vi "Update.vi"(8 "error in (no error)":errorcluster, 11 "Deck in":refnum<class "Deck.lvclass">) -> (0 "error out":errorcluster, 2 "Audio Block":dbl[][](array[numeric]), 3 "Deck out":refnum<class "Deck.lvclass">)   [LabVIEW 2019, in "Deck.lvclass"]
uses:
  Deck.lvclass
  Deck.lvclass/Deck.ctl
  State.ctl
  Packed Libraries/Globals.lvlibp/Constants.vi
  <vilib>/gmath/NI_Gmath.lvlib
  Libraries/User Interface/User Interface.lvlib
  Packed Libraries/Messaging.lvlibp
  Packed Libraries/Globals.lvlibp
  Packed Libraries/Audio Processing.lvlibp
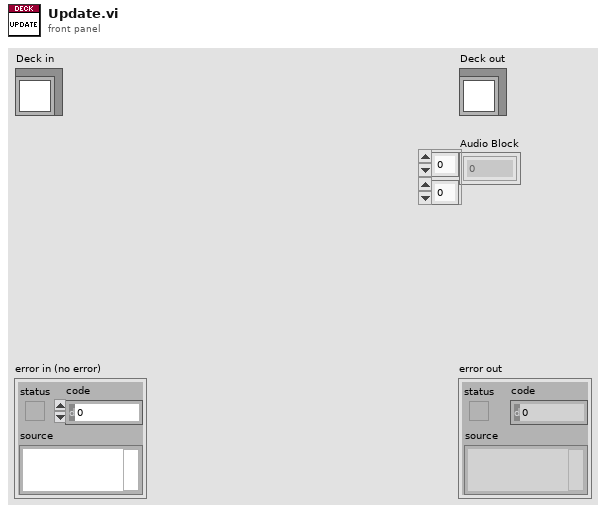
[diagram p1: front panel]
types:
  T1 = typedef "Deck.lvclass/State.ctl" = enum16{"No Track", "Loading", "Active", "Scratching", "Brake", "Backspin"}
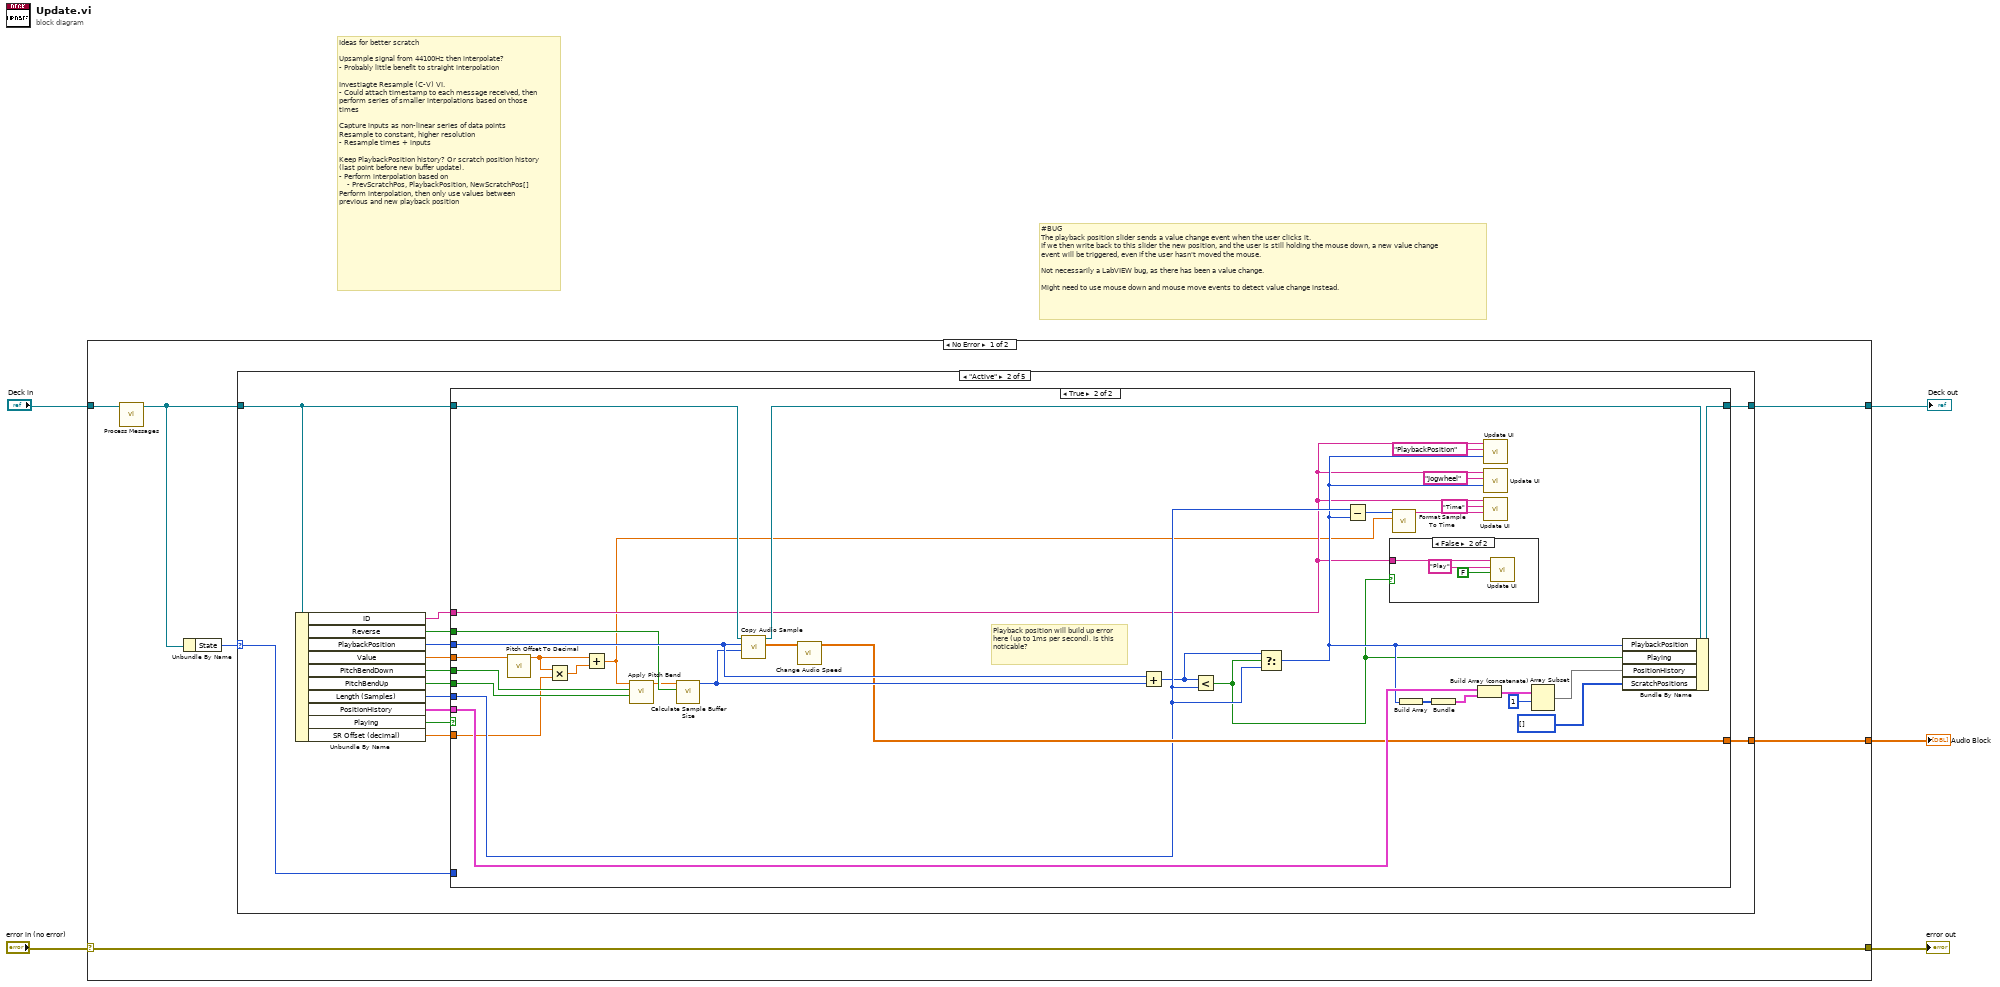
[diagram p0: block diagram]
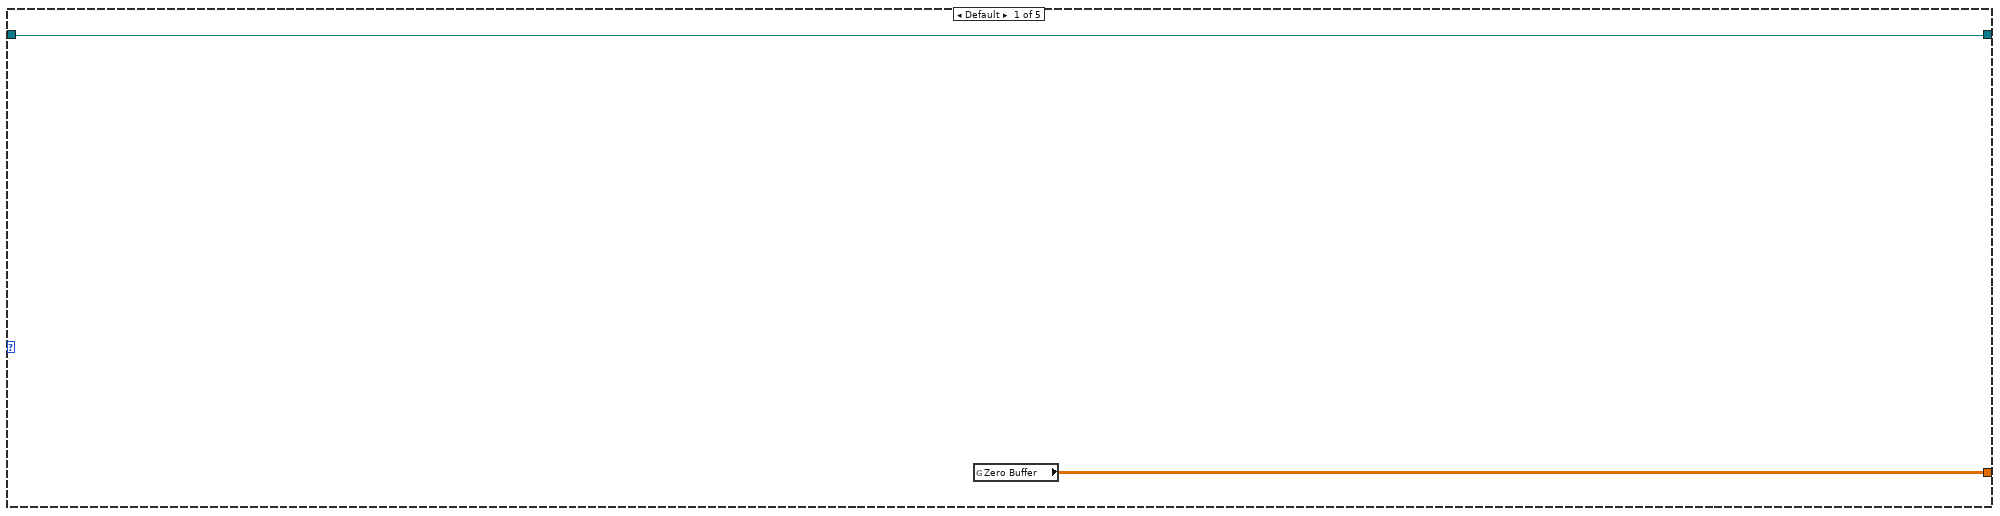
[diagram p2: hidden frame]
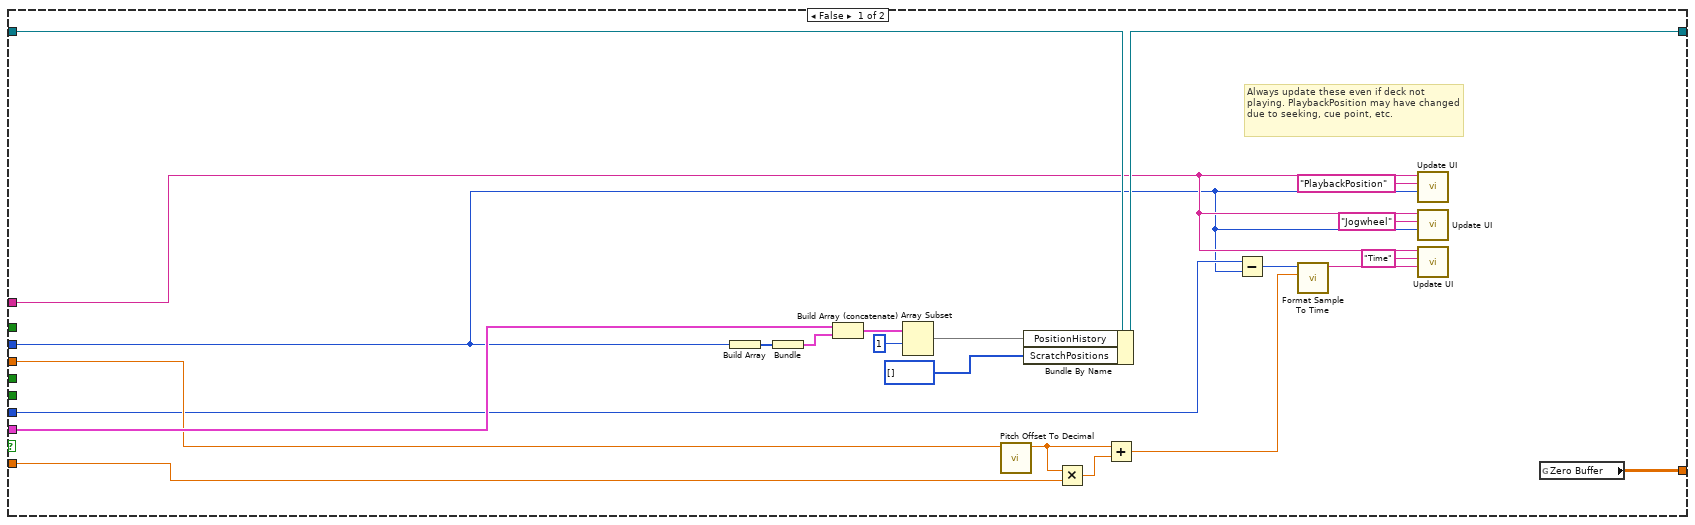
[diagram p3: hidden frame]
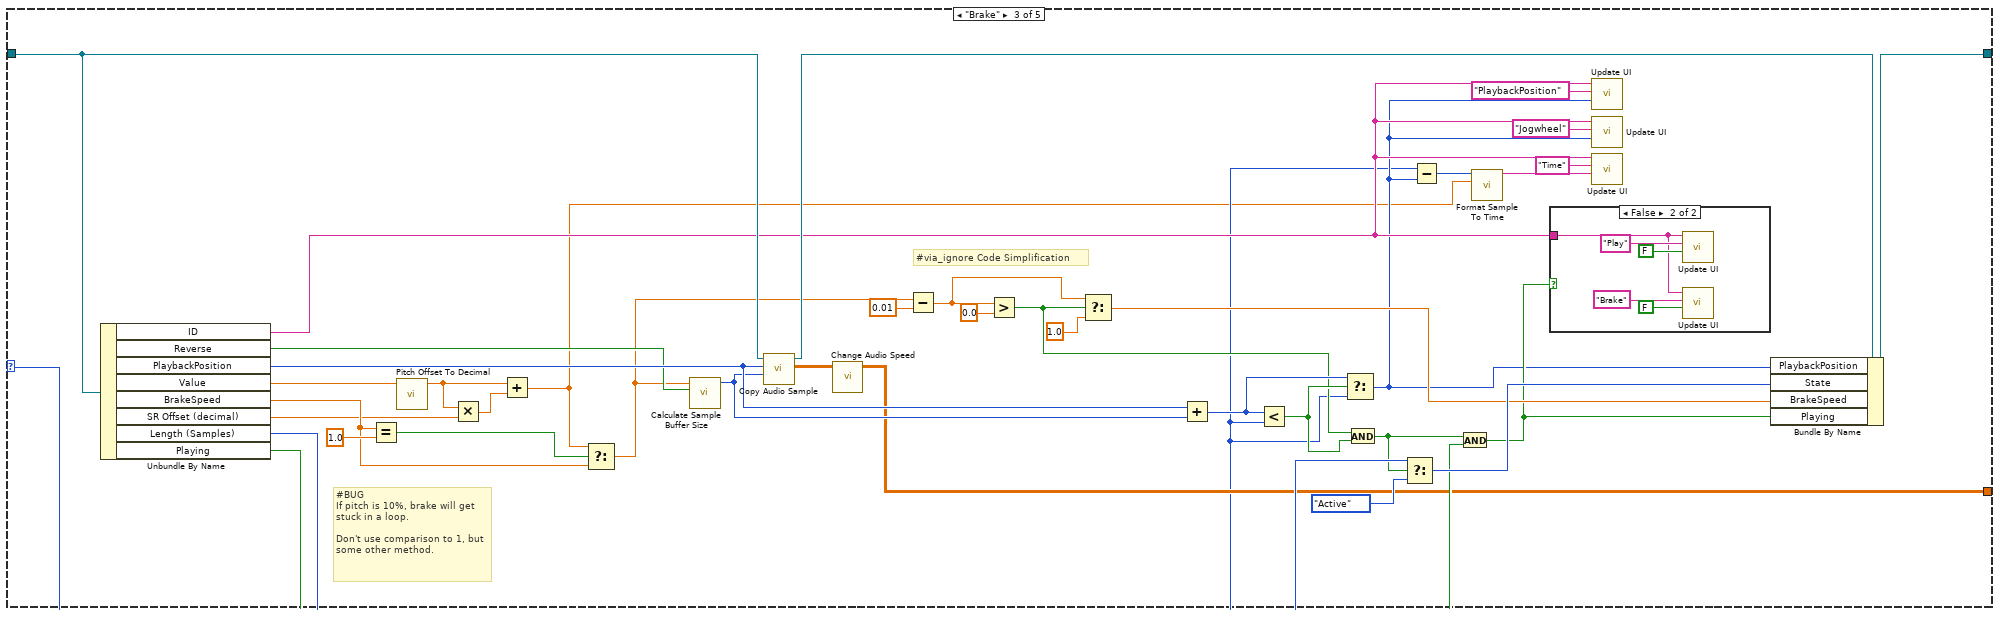
[diagram p5: hidden frame]
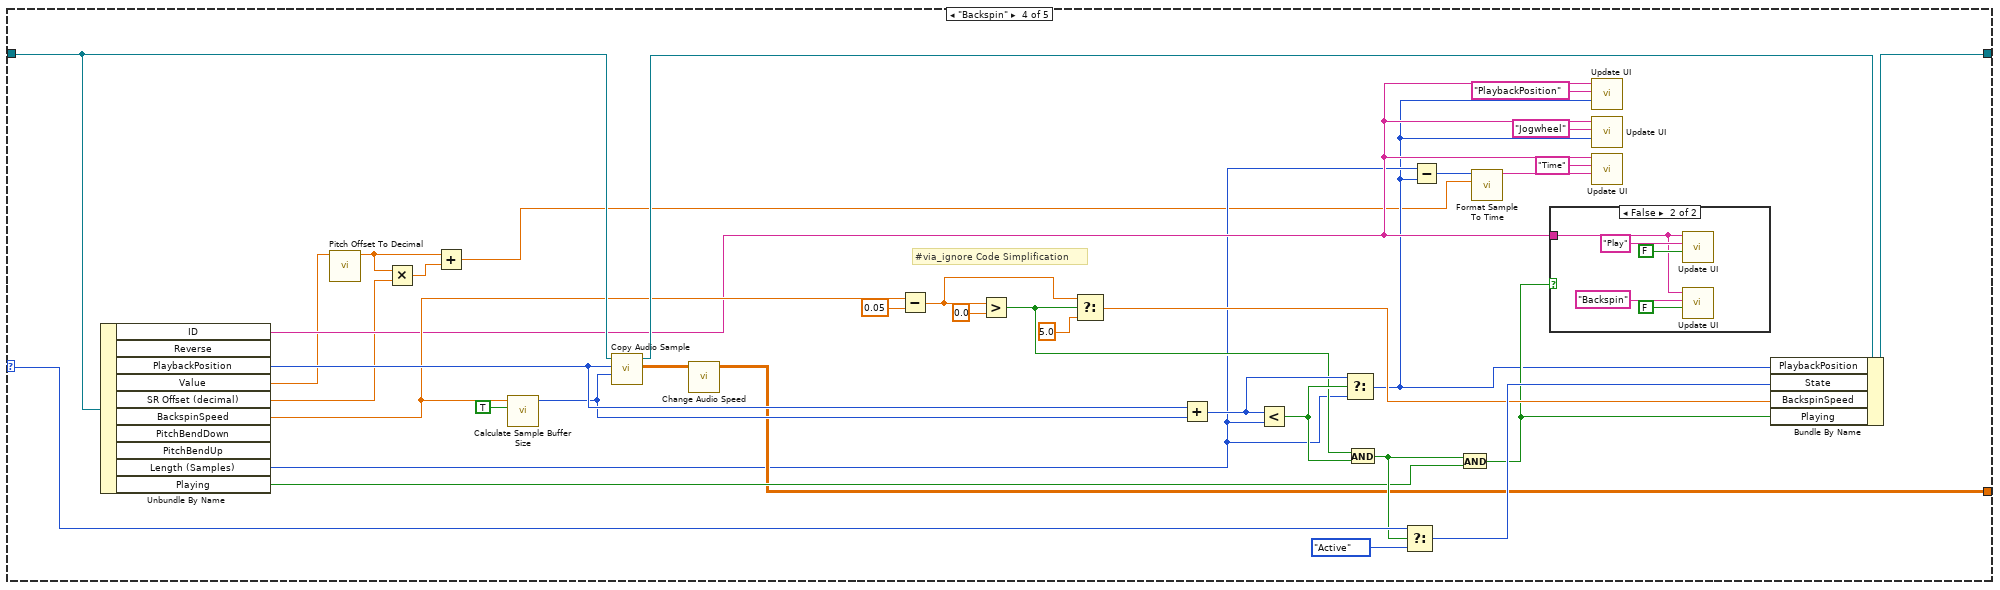
[diagram p7: hidden frame]
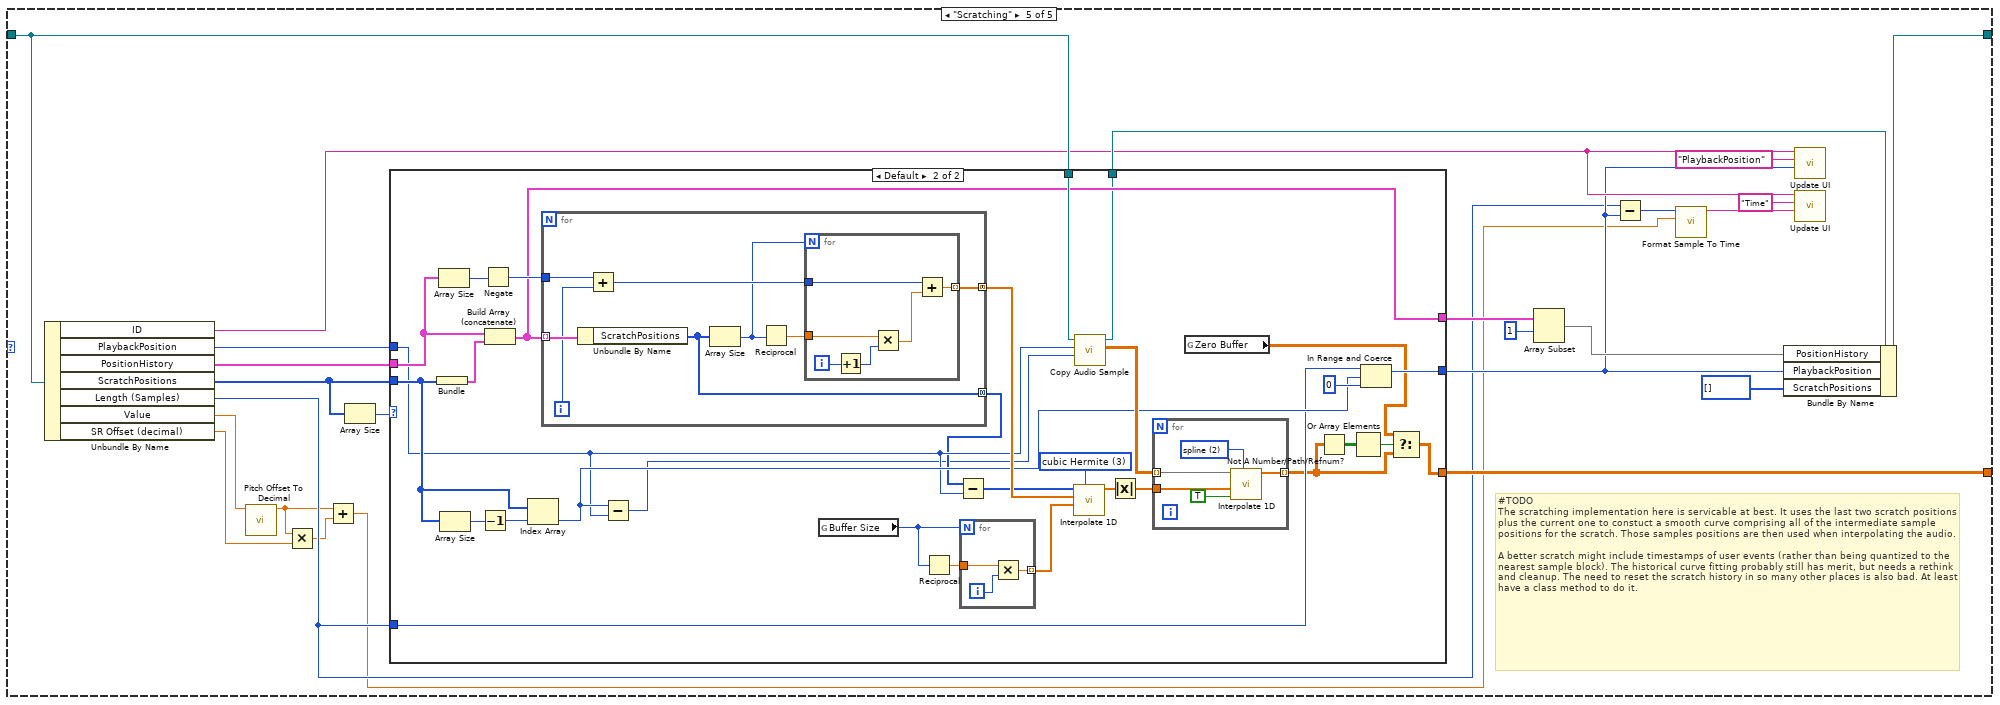
[diagram p9: hidden frame]
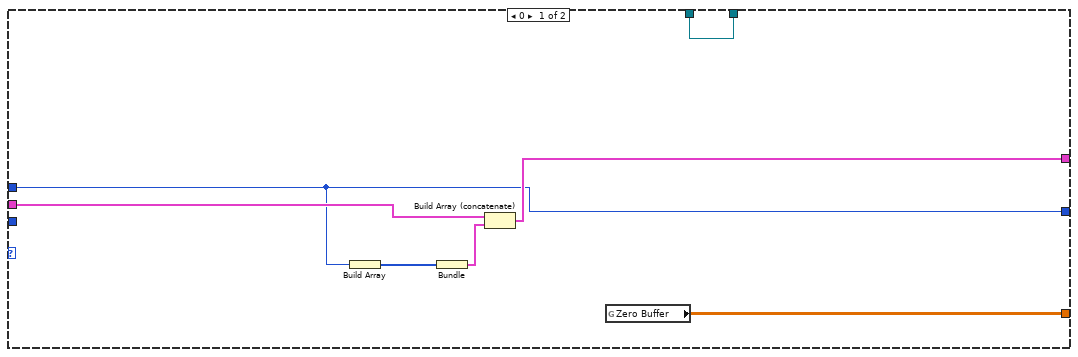
[diagram p10: hidden frame]
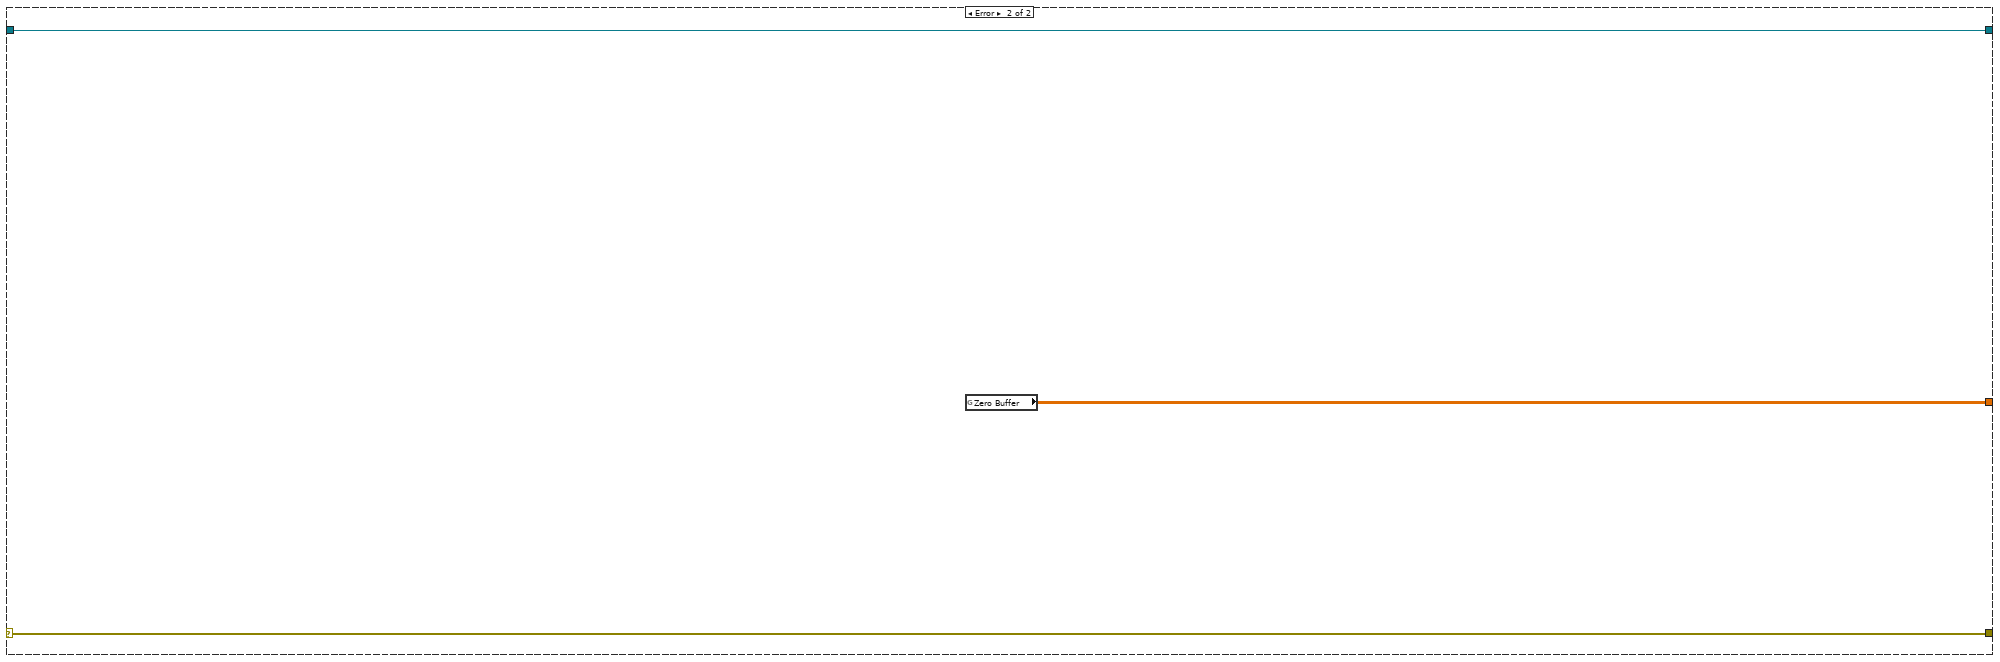
[diagram p11: hidden frame]
diagram:
  # "Ideas for better scratch\n\nUpsample signal from 44100Hz then interpolate?\n- Probably little benefit to straight interpolation\n\nInvestiagte Resample (C-V) VI.\n- Could attach timestamp to each message received, then perform series of smaller interpolations based on those times\n\nCapture inputs as non-linear series of data points\nResample to constant, higher resolution\n- Resample times + inputs\n\nKeep PlaybackPosition history? Or scratch position history (last point before new buffer update).\n- Perform interpolation based on\n    - PrevScratchPos, PlaybackPosition, NewScratchPos[]\nPerform interpolation, then only use values between previous and new playback position"
  # "#BUG\nThe playback position slider sends a value change event when the user clicks it.\nIf we then write back to this slider the new position, and the user is still holding the mouse down, a new value change event will be triggered, even if the user hasn't moved the mouse.\n\nNot necessarily a LabVIEW bug, as there has been a value change.\n\nMight need to use mouse down and mouse move events to detect value change instead."
  n1 = case shown="No Error" "error in (no error)" {
    selector: "error in (no error)" -> [w11 w258]
    tunnel: [w11 w258] -> w4
    tunnel: [w9 w257] -> w2
    tunnel: "Deck in" -> [w6 w257]
    tunnel: [w8 w256] -> w1
    frame No Error {
      n2 = call "Process Messages.vi"("Deck in"=w6) -> ("Deck out"=w7:refnum<class "Deck.lvclass">)  [unwired: 9 in, 1 out]
      n3 = Unbundle By Name(w7) -> ("State"=w10:T1)
      n4 = case shown="\"Active\"" w10 {
        selector: w10 -> [_ w20 w120 w161 _]
        tunnel: [w13 w27 w125 w166 w195] -> w9
        tunnel: w7 -> [w13 w26 w123 w164 w193]
        tunnel: [w12 w24 w99 w145 w184] -> w8
        frame Default {
          n5 = global read "Constants.vi" "Zero Buffer"() -> (w12:dbl[][])
        }
        frame "Active" {
          n6 = Unbundle By Name(w26) -> ("ID"=w16:string, "Reverse"=w15:bool, "PlaybackPosition"=w25:i32, "Value"=w22:dbl, "PitchBendDown"=w23:bool, "PitchBendUp"=w21:bool, "Length (Samples)"=w18:i32, "PositionHistory"=w19:cluster{"Positions":i32[]}[], "Playing"=w17:bool, "SR Offset (decimal)"=w14:dbl)
          n7 = case shown="True" w17 {
            tunnel: [w43 w83] -> w27
            tunnel: w26 -> [w42 w81]
            tunnel: w25 -> [w29 w80]
            tunnel: [w50 w68] -> w24
            tunnel: w23 -> [_ w54]
            tunnel: w22 -> [w33 w72]
            tunnel: w21 -> [_ w55]
            tunnel: w20 -> [_ _]
            tunnel: w19 -> [w41 w77]
            tunnel: w16 -> [w31 w58]
            tunnel: w18 -> [w30 w67]
            tunnel: w15 -> [_ w71]
            tunnel: w14 -> [w32 w53]
            frame False {
              # "Always update these even if deck not playing. PlaybackPosition may have changed due to seeking, cue point, etc."
              n8 = Build Array(w29) -> (w46:i32[])
              n9 = Bundle(w46) -> (w45:cluster{i32[]})  [unwired: 1 in]
              n10 = Build Array (concatenate)(w41, w45) -> (w49:cluster{"Positions":i32[]}[])
              n11 = Array Subset(array=w49, index=1) -> (w47:cluster{"Positions":i32[]}[])  [unwired: 1 in]
              n12 = call "Pitch Offset To Decimal.vi"("Pitch Offset (%)"=w33) -> ("Pitch (decimal)"=w34:dbl)  [unwired: 10 in]
              n13 = Bundle By Name(cluster=w42, "PositionHistory"=w47, "ScratchPositions"=i32[] []) -> (w43:refnum<class "Deck.lvclass">)
              n14 = Multiply(x=w34, y=w32) -> (x*y=w35:dbl)
              n15 = Add(x=w34, y=w35) -> (x+y=w28:dbl)
              n16 = Subtract(x=w30, y=w29) -> (x-y=w40:i32)
              n17 = call "Format Sample To Time.vi"("Pitch (decimal) (1)"=w28, "Samples"=w40) -> ("Formatted Time"=w37:string)  [unwired: 9 in]
              n18 = call "Update UI.vi"("Data"=w29, "Target"="PlaybackPosition" ("format string"), "ID"=w31) -> ()  [unwired: 8 in, 1 out]
              n19 = call "Update UI.vi"("Data"=w29, "Target"="Jogwheel" ("format string"), "ID"=w31) -> ()  [unwired: 8 in, 1 out]
              n20 = call "Update UI.vi"("Data"=w37, "Target"="Time" ("format string"), "ID"=w31) -> ()  [unwired: 8 in, 1 out]
              n21 = global read "Constants.vi" "Zero Buffer"() -> (w50:dbl[][])
            }
            frame True {
              # "Playback position will build up error here (up to 1ms per second). Is this noticable?"
              n22 = call "Pitch Offset To Decimal.vi"("Pitch Offset (%)"=w72) -> ("Pitch (decimal)"=w52:dbl)  [unwired: 10 in]
              n23 = Multiply(x=w52, y=w53) -> (x*y=w51:dbl)
              n24 = Add(x=w52, y=w51) -> (x+y=w57:dbl)
              n25 = call "Apply Pitch Bend.vi"("Pitch Bend Up (F)"=w55, "Pitch Bend Down (F)"=w54, "Pitch (decimal) In"=w57) -> ("Pitch (decimal) Out"=w56:dbl)  [unwired: 8 in]
              n26 = call "Calculate Sample Buffer Size.vi"("Reverse (F)"=w71, "Speed Multiplier"=w56) -> ("Sample Size"=w70:i32)  [unwired: 9 in]
              n27 = call "Copy Audio Sample.vi"("Length"=w70, "Offset"=w80, "Deck in"=w81) -> ("Audio Block"=w69:dbl[][], "Deck out"=w82:refnum<class "Deck.lvclass">)  [unwired: 6 in, 1 out]
              n28 = call "Change Audio Speed.vi"("Audio Block"=w69) -> ("Interpolated Audio"=w68:dbl[][])  [unwired: 10 in]
              n29 = Add(x=w80, y=w70) -> (x+y=w66:i32)
              n30 = Less?(x=w66, y=w67) -> (x < y?=w59:bool)
              n31 = Select(t=w66, s=w59, f=w67) -> (s? t:f=w62:i32)
              n32 = Subtract(x=w67, y=w62) -> (x-y=w65:i32)
              n33 = case shown="False" w59 {
                tunnel: w58 -> [_ w84]
                frame True {
                }
                frame False {
                  n34 = call "Update UI.vi"("Data"=FALSE, "Target"="Play" ("format string"), "ID"=w84) -> ()  [unwired: 8 in, 1 out]
                }
              }
              n35 = call "Format Sample To Time.vi"("Pitch (decimal) (1)"=w57, "Samples"=w65) -> ("Formatted Time"=w61:string)  [unwired: 9 in]
              n36 = Build Array(w62) -> (w75:i32[])
              n37 = Bundle(w75) -> (w74:cluster{i32[]})  [unwired: 1 in]
              n38 = Build Array (concatenate)(w77, w74) -> (w79:cluster{"Positions":i32[]}[])
              n39 = call "Update UI.vi"("Data"=w62, "Target"="PlaybackPosition" ("format string"), "ID"=w58) -> ()  [unwired: 8 in, 1 out]
              n40 = call "Update UI.vi"("Data"=w62, "Target"="Jogwheel" ("format string"), "ID"=w58) -> ()  [unwired: 8 in, 1 out]
              n41 = call "Update UI.vi"("Data"=w61, "Target"="Time" ("format string"), "ID"=w58) -> ()  [unwired: 8 in, 1 out]
              n42 = Array Subset(array=w79, index=1) -> (w76:cluster{"Positions":i32[]}[])  [unwired: 1 in]
              n43 = Bundle By Name(cluster=w82, "PlaybackPosition"=w62, "Playing"=w59, "PositionHistory"=w76, "ScratchPositions"=i32[] []) -> (w83:refnum<class "Deck.lvclass">)
            }
          }
        }
        frame "Brake" {
          # "#via_ignore Code Simplification"
          # "#BUG\nIf pitch is 10%, brake will get stuck in a loop.\n\nDon't use comparison to 1, but some other method."
          n44 = Unbundle By Name(w123) -> ("ID"=w93:string, "Reverse"=w102:bool, "PlaybackPosition"=w122:i32, "Value"=w104:dbl, "BrakeSpeed"=w108:dbl, "SR Offset (decimal)"=w88:dbl, "Length (Samples)"=w91:i32, "Playing"=w106:bool)
          n45 = Equal?(x=w108, y=1.0) -> (x = y?=w109:bool)
          n46 = call "Pitch Offset To Decimal.vi"("Pitch Offset (%)"=w104) -> ("Pitch (decimal)"=w89:dbl)  [unwired: 10 in]
          n47 = Multiply(x=w89, y=w88) -> (x*y=w90:dbl)
          n48 = Add(x=w89, y=w90) -> (x+y=w87:dbl)
          n49 = Select(t=w87, s=w109, f=w108) -> (s? t:f=w101:dbl)
          n50 = call "Calculate Sample Buffer Size.vi"("Reverse (F)"=w102, "Speed Multiplier"=w101) -> ("Sample Size"=w100:i32)  [unwired: 9 in]
          n51 = call "Copy Audio Sample.vi"("Length"=w100, "Offset"=w122, "Deck in"=w123) -> ("Audio Block"=w103:dbl[][], "Deck out"=w124:refnum<class "Deck.lvclass">)  [unwired: 6 in, 1 out]
          n52 = call "Change Audio Speed.vi"("Audio Block"=w103) -> ("Interpolated Audio"=w99:dbl[][])  [unwired: 10 in]
          n53 = Subtract(x=w101, y=0.01) -> (x-y=w111:dbl)
          n54 = Greater?(x=w111, y=0.0) -> (0:w114:bool)
          n55 = Select(t=w111, s=w114, f=1.0 ("t")) -> (s? t:f=w113:dbl)
          n56 = Add(x=w122, y=w100) -> (x+y=w121:i32)
          n57 = Less?(x=w121, y=w91) -> (x < y?=w115:bool)
          n58 = Select(t=w121, s=w115, f=w91) -> (s? t:f=w92:i32)
          n59 = And(x=w114, y=w115) -> (x .and. y?=w107:bool)
          n60 = Select(t=w120, s=w107, f=State."Active") -> (s? t:f=w119:T1)
          n61 = Subtract(x=w91, y=w92) -> (x-y=w98:i32)
          n62 = And(x=w107, y=w106) -> (x .and. y?=w105:bool)
          n63 = call "Format Sample To Time.vi"("Pitch (decimal) (1)"=w87, "Samples"=w98) -> ("Formatted Time"=w95:string)  [unwired: 9 in]
          n64 = case shown="False" w105 {
            tunnel: w93 -> [_ w126]
            frame True {
            }
            frame False {
              n65 = call "Update UI.vi"("Data"=FALSE, "Target"="Play" ("format string"), "ID"=w126) -> ()  [unwired: 8 in, 1 out]
              n66 = call "Update UI.vi"("Data"=FALSE, "Target"="Brake" ("format string"), "ID"=w126) -> ()  [unwired: 8 in, 1 out]
            }
          }
          n67 = call "Update UI.vi"("Data"=w92, "Target"="PlaybackPosition" ("format string"), "ID"=w93) -> ()  [unwired: 8 in, 1 out]
          n68 = call "Update UI.vi"("Data"=w92, "Target"="Jogwheel" ("format string"), "ID"=w93) -> ()  [unwired: 8 in, 1 out]
          n69 = call "Update UI.vi"("Data"=w95, "Target"="Time" ("format string"), "ID"=w93) -> ()  [unwired: 8 in, 1 out]
          n70 = Bundle By Name(cluster=w124, "PlaybackPosition"=w92, "State"=w119, "BrakeSpeed"=w113, "Playing"=w105) -> (w125:refnum<class "Deck.lvclass">)
        }
        frame "Backspin" {
          # "#via_ignore Code Simplification"
          n71 = Unbundle By Name(w164) -> ("ID"=w139:string, "PlaybackPosition"=w163:i32, "Value"=w135:dbl, "SR Offset (decimal)"=w133:dbl, "BackspinSpeed"=w149:dbl, "Length (Samples)"=w137:i32, "Playing"=w150:bool)  [unwired: 3 out]
          n72 = call "Pitch Offset To Decimal.vi"("Pitch Offset (%)"=w135) -> ("Pitch (decimal)"=w131:dbl)  [unwired: 10 in]
          n73 = Multiply(x=w131, y=w133) -> (x*y=w134:dbl)
          n74 = Add(x=w131, y=w134) -> (x+y=w132:dbl)
          n75 = call "Calculate Sample Buffer Size.vi"("Reverse (F)"=TRUE, "Speed Multiplier"=w149) -> ("Sample Size"=w147:i32)  [unwired: 9 in]
          n76 = call "Copy Audio Sample.vi"("Length"=w147, "Offset"=w163, "Deck in"=w164) -> ("Audio Block"=w146:dbl[][], "Deck out"=w165:refnum<class "Deck.lvclass">)  [unwired: 6 in, 1 out]
          n77 = call "Change Audio Speed.vi"("Audio Block"=w146) -> ("Interpolated Audio"=w145:dbl[][])  [unwired: 10 in]
          n78 = Subtract(x=w149, y=0.05) -> (x-y=w152:dbl)
          n79 = Greater?(x=w152, y=0.0) -> (0:w155:bool)
          n80 = Select(t=w152, s=w155, f=5.0 ("t")) -> (s? t:f=w154:dbl)
          n81 = Add(x=w163, y=w147) -> (x+y=w162:i32)
          n82 = Less?(x=w162, y=w137) -> (x < y?=w156:bool)
          n83 = Select(t=w162, s=w156, f=w137) -> (s? t:f=w136:i32)
          n84 = And(x=w155, y=w156) -> (x .and. y?=w151:bool)
          n85 = Select(t=w161, s=w151, f=State."Active") -> (s? t:f=w160:T1)
          n86 = Subtract(x=w137, y=w136) -> (x-y=w144:i32)
          n87 = And(x=w151, y=w150) -> (x .and. y?=w138:bool)
          n88 = call "Format Sample To Time.vi"("Pitch (decimal) (1)"=w132, "Samples"=w144) -> ("Formatted Time"=w141:string)  [unwired: 9 in]
          n89 = case shown="False" w138 {
            tunnel: w139 -> [_ w167]
            frame True {
            }
            frame False {
              n90 = call "Update UI.vi"("Data"=FALSE, "Target"="Play" ("format string"), "ID"=w167) -> ()  [unwired: 8 in, 1 out]
              n91 = call "Update UI.vi"("Data"=FALSE, "Target"="Backspin" ("format string"), "ID"=w167) -> ()  [unwired: 8 in, 1 out]
            }
          }
          n92 = call "Update UI.vi"("Data"=w136, "Target"="PlaybackPosition" ("format string"), "ID"=w139) -> ()  [unwired: 8 in, 1 out]
          n93 = call "Update UI.vi"("Data"=w136, "Target"="Jogwheel" ("format string"), "ID"=w139) -> ()  [unwired: 8 in, 1 out]
          n94 = call "Update UI.vi"("Data"=w141, "Target"="Time" ("format string"), "ID"=w139) -> ()  [unwired: 8 in, 1 out]
          n95 = Bundle By Name(cluster=w165, "PlaybackPosition"=w136, "State"=w160, "BackspinSpeed"=w154, "Playing"=w138) -> (w166:refnum<class "Deck.lvclass">)
        }
        frame "Scratching" {
          # "#TODO\nThe scratching implementation here is servicable at best. It uses the last two scratch positions plus the current one to constuct a smooth curve comprising all of the intermediate sample positions for the scratch. Those samples positions are then used when interpolating the audio.\n\nA better scratch might include timestamps of user events (rather than being quantized to the nearest sample block). The historical curve fitting probably still has merit, but needs a rethink and cleanup. The need to reset the scratch history in so many other places is also bad. At least have a class method to do it."
          n96 = Unbundle By Name(w193) -> ("ID"=w179:string, "PlaybackPosition"=w192:i32, "PositionHistory"=w191:cluster{"Positions":i32[]}[], "ScratchPositions"=w189:i32[], "Length (Samples)"=w177:i32, "Value"=w176:dbl, "SR Offset (decimal)"=w174:dbl)
          n97 = call "Pitch Offset To Decimal.vi"("Pitch Offset (%)"=w176) -> ("Pitch (decimal)"=w172:dbl)  [unwired: 10 in]
          n98 = Multiply(x=w172, y=w174) -> (x*y=w175:dbl)
          n99 = Add(x=w172, y=w175) -> (x+y=w173:dbl)
          n100 = Array Size(array=w189) -> (size(s)=w190:i32)
          n101 = case shown="Default" w190 {
            tunnel: [w198 w232] -> w178
            tunnel: [w202 w209] -> w194
            tunnel: w193 -> [w202 w233]
            tunnel: w192 -> [w198 w215]
            tunnel: [w196 w205] -> w184
            tunnel: w177 -> [_ w211]
            tunnel: w191 -> [w199 w225]
            tunnel: [w200 w216] -> w188
            tunnel: w189 -> [_ w221]
            frame 0 {
              n102 = Build Array(w198) -> (w197:i32[])
              n103 = Bundle(w197) -> (w201:cluster{i32[]})  [unwired: 1 in]
              n104 = Build Array (concatenate)(w199, w201) -> (w200:cluster{"Positions":i32[]}[])
              n105 = global read "Constants.vi" "Zero Buffer"() -> (w196:dbl[][])
            }
            frame Default {
              w227 = 3 items=["nearest", "linear", "spline", "cubic Hermite", "Lagrange"] ("method")
              n106 = Bundle("ScratchPositions"=w221) -> (w226:cluster{"ScratchPositions":i32[]})  [unwired: 1 in]
              n107 = Array Size(array=w225) -> (size(s)=w229:i32)
              n108 = Array Size(array=w221) -> (size(s)=w223:i32)
              n109 = Decrement(x=w223) -> (x-1=w222:i32)
              n110 = Negate(x=w229) -> (-x=w228:i32)
              n111 = Build Array (concatenate)(w225, w226) -> (w216:cluster{"ScratchPositions":i32[]}[])
              n112 = Index Array(array=w221, index=w222) -> (element=w217:i32)
              n113 = for {
                tunnel: w216 -> [w244] mode=indexing
                tunnel: w228 -> [w238]
                tunnel: [w242] -> w224 mode=concatenating
                tunnel: [w241] -> w213 mode=concatenating
                i -> [w240]
                n114 = Unbundle By Name(w244) -> ("ScratchPositions"=w241:i32[])
                n115 = Add(x=w238, y=w240) -> (x+y=w239:i32)
                n116 = Array Size(array=w241) -> (size(s)=w237:i32)
                n117 = Reciprocal(x=w237) -> (1/x=w243:dbl)
                n118 = for {
                  N: w237 -> [_]
                  tunnel: w243 -> [w247]
                  tunnel: w239 -> [w250]
                  tunnel: [w246] -> w242 mode=indexing
                  i -> [w249]
                  n119 = Increment(x=w249) -> (x+1=w245:i32)
                  n120 = Multiply(x=w247, y=w245) -> (x*y=w248:dbl)
                  n121 = Add(x=w250, y=w248) -> (x+y=w246:dbl)
                }
              }
              n122 = Subtract(x=w217, y=w215) -> (x-y=w210:i32)
              n123 = global read "Constants.vi" "Buffer Size"() -> (w204:i32)
              n124 = Reciprocal(x=w204) -> (1/x=w220:dbl)
              n125 = Subtract(x=w213, y=w215) -> (x-y=w214:i32[])
              n126 = for {
                N: w204 -> [_]
                tunnel: w220 -> [w235]
                tunnel: [w234] -> w219 mode=indexing
                i -> [w236]
                n127 = Multiply(x=w235, y=w236) -> (x*y=w234:dbl)
              }
              n128 = call <vilib>:"Interpolate 1D.vi"("method"=w227, "xi"=w219, "X"=w224, "Y"=w214) -> ("yi"=w218:dbl[])  [unwired: 5 in, 2 out]
              n129 = call "Copy Audio Sample.vi"("Length"=w210, "Offset"=w215, "Deck in"=w233) -> ("Audio Block"=w231:dbl[][], "Deck out"=w209:refnum<class "Deck.lvclass">)  [unwired: 6 in, 1 out]
              n130 = Absolute Value(x=w218) -> (abs(x)=w212:dbl[])
              n131 = for {
                tunnel: w231 -> [w251] mode=indexing
                tunnel: w212 -> [w252]
                tunnel: [w253] -> w206 mode=indexing
                w254 = 2 items=["nearest", "linear", "spline", "cubic Hermite", "Lagrange"] ("method")
                n132 = call <vilib>:"Interpolate 1D.vi"("method"=w254, "X is monotonic"=TRUE, "xi"=w252, "Y"=w251) -> ("yi"=w253:dbl[])  [unwired: 5 in, 2 out]
              }
              n133 = global read "Constants.vi" "Zero Buffer"() -> (w203:dbl[][])
              n134 = Not A Number/Path/Refnum?(number/path/refnum=w206) -> (NaN/Path/Refnum?=w208:bool[][])
              n135 = Or Array Elements(Boolean array=w208) -> (logical OR=w207:bool)
              n136 = In Range and Coerce(upper limit=w211, x=w217, lower limit=0) -> (coerced(x)=w232:i32)  [unwired: 1 out]
              n137 = Select(t=w203, s=w207, f=w206) -> (s? t:f=w205:dbl[][])
            }
          }
          n138 = Array Subset(array=w188, index=1) -> (w186:cluster{"ScratchPositions":i32[]}[])  [unwired: 1 in]
          n139 = Subtract(x=w177, y=w178) -> (x-y=w183:i32)
          n140 = call "Format Sample To Time.vi"("Pitch (decimal) (1)"=w173, "Samples"=w183) -> ("Formatted Time"=w181:string)  [unwired: 9 in]
          n141 = Bundle By Name(cluster=w194, "PositionHistory"=w186, "PlaybackPosition"=w178, "ScratchPositions"=i32[] []) -> (w195:refnum<class "Deck.lvclass">)
          n142 = call "Update UI.vi"("Data"=w178, "Target"="PlaybackPosition" ("format string"), "ID"=w179) -> ()  [unwired: 8 in, 1 out]
          n143 = call "Update UI.vi"("Data"=w181, "Target"="Time" ("format string"), "ID"=w179) -> ()  [unwired: 8 in, 1 out]
        }
      }
    }
    frame Error {
      n144 = global read "Constants.vi" "Zero Buffer"() -> (w256:dbl[][])
    }
  }
  "error out" <- w4
  "Deck out" <- w2
  "Audio Block" <- w1
